vi "SCAN IM Stage Engine.vi"(0 "Notifier Name":string, 11 "COM Port":string[](array[string])) -> ()   [LabVIEW 2016]
uses:
  Stages Controls/Stage XY Control.ctl
  Stages Controls/Stage Status.ctl
  Stages Controls/Stage Notifier Element.ctl
  Stages Controls/Stage Actions.ctl
  <userlib>/Tango_DLL/Tango_DLL.lvlib
panel:
  out "Status":T1
  in  "Quit":bool
  in  "XY Control":T2
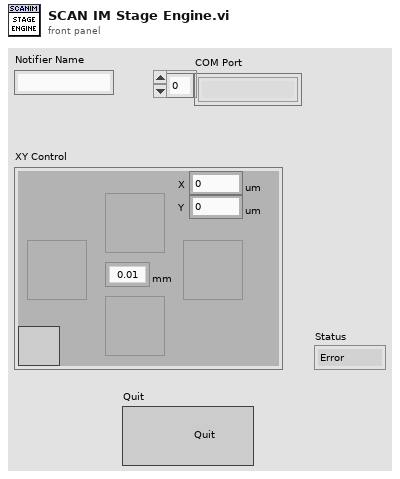
[diagram p1: front panel]
types:
  T1 = typedef "Stage Status.ctl" = enum16{"Error", "Abort", "Busy", "On Target"}
  T2 = typedef "Stage XY Control.ctl" = cluster{"Left":bool, "Right":bool, "Up":bool, "Down":bool, "Home":bool, "StageStep":enum16{"0.01", "0.02", "0.05", "0.1", "0.5", "1", "2", "5", "10", "20", "50", "100", "500", "1000", "2000", "5000"}, "Y":dbl, "X":dbl}
  T3 = typedef "Stage Notifier Element.ctl" = cluster{"Action":T4, "Axis":bool[], "Setpoint":dbl[], "Velocity":dbl, "Cmd Recvd?":bool, "Position":dbl[], "Status":T1, "Misc":variant}
  T4 = typedef "Stage Actions.ctl" = enum16{"Get Position", "MVR", "MOVE", "HALT", "ONTARGET", "ERROR", "REFERENCE", "INIT", "VELOCITY", "STATUS", "EXIT", "HOME", "ZEROPOS", "NANOPOS", "ANALOG", "QUIT"}
  T5 = cluster{"Left":bool, "Right":bool, "Up":bool, "Down":bool, "Home":bool, "StageStep":bool, "Y":bool, "X":bool}
  T6 = enum16{"0.01", "0.02", "0.05", "0.1", "0.5", "1", "2", "5", "10", "20", "50", "100", "500", "1000", "2000", "5000"}
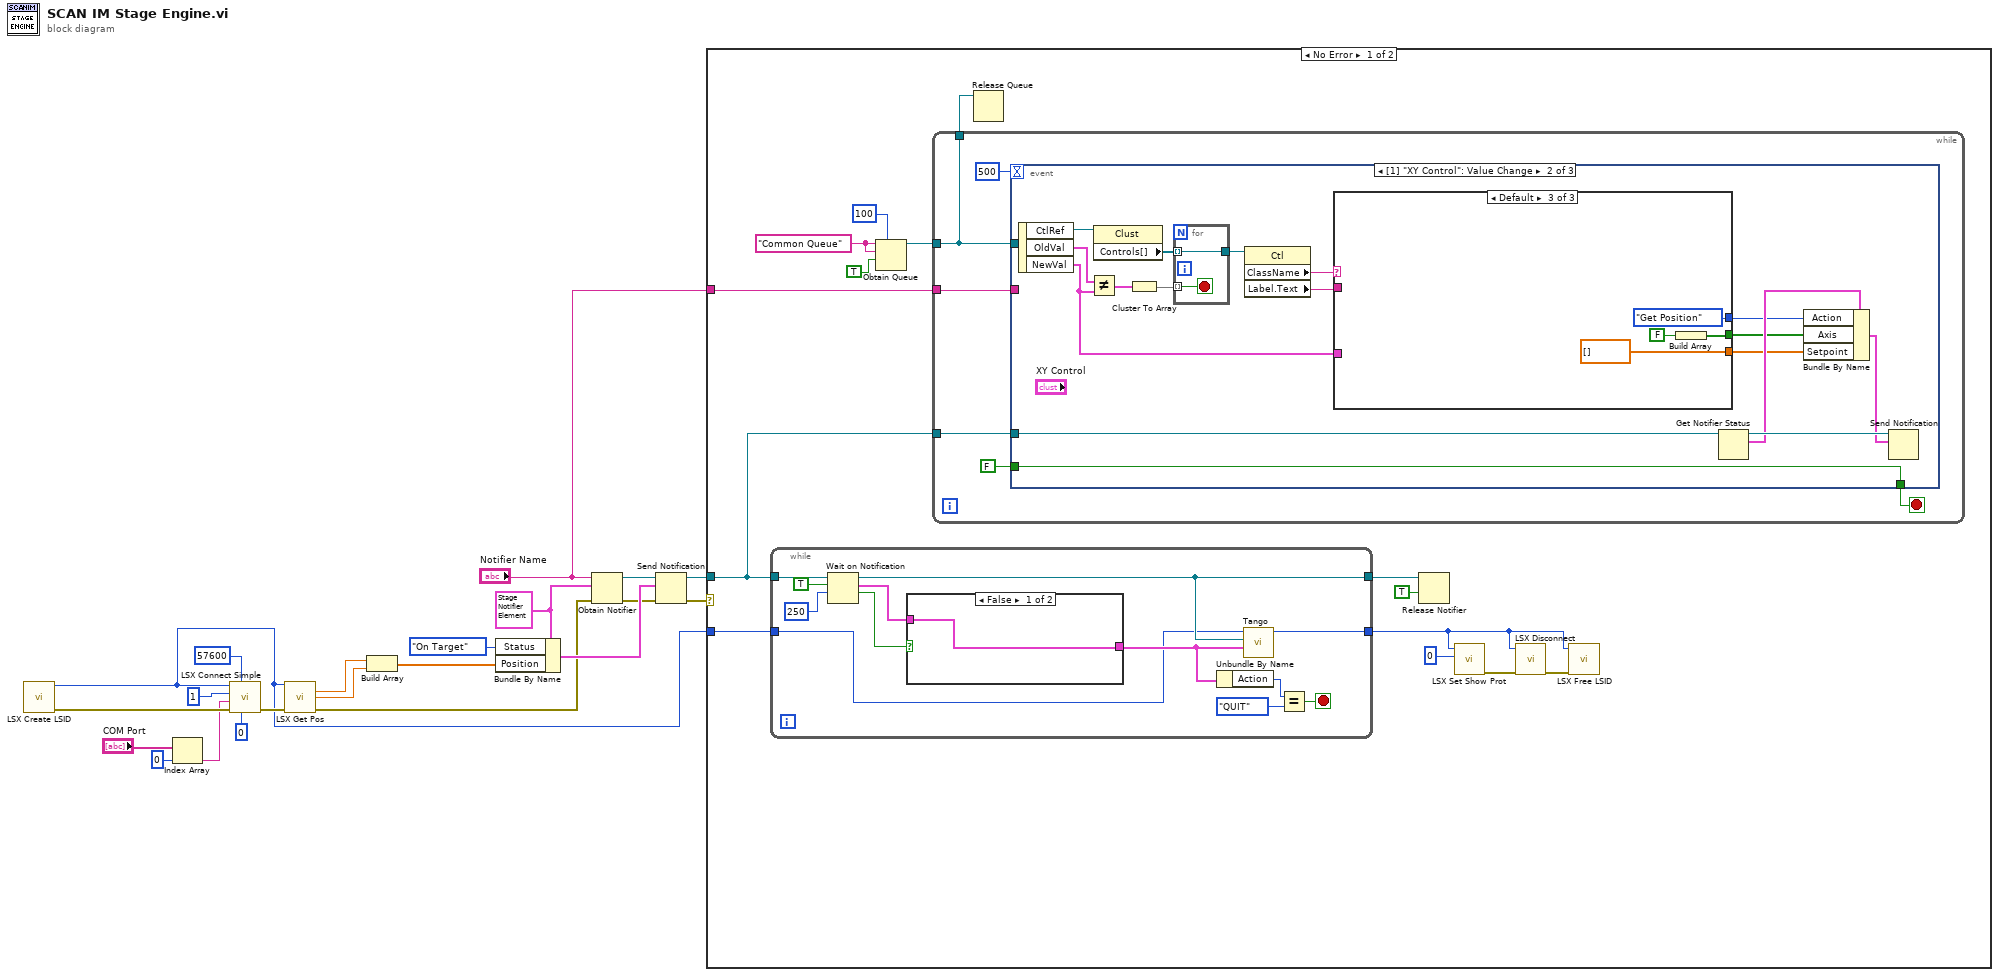
[diagram p0: block diagram]
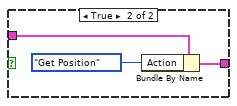
[diagram p2: hidden frame]
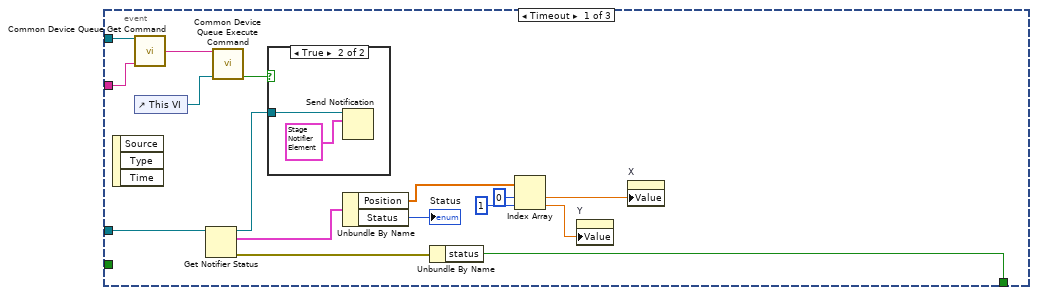
[diagram p3: hidden frame]
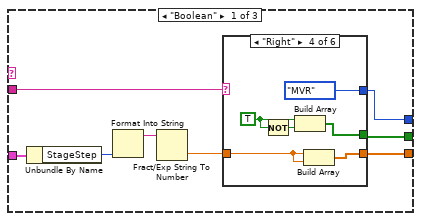
[diagram p5: hidden frame]
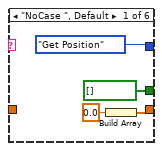
[diagram p6: hidden frame]
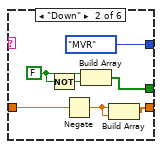
[diagram p7: hidden frame]
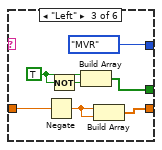
[diagram p8: hidden frame]
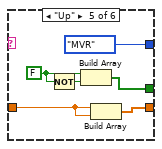
[diagram p9: hidden frame]
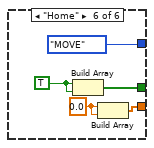
[diagram p10: hidden frame]
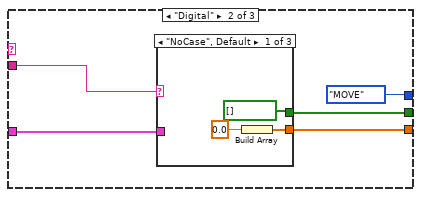
[diagram p11: hidden frame]
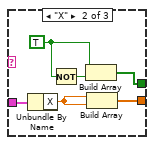
[diagram p12: hidden frame]
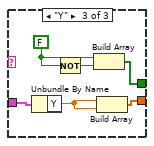
[diagram p13: hidden frame]
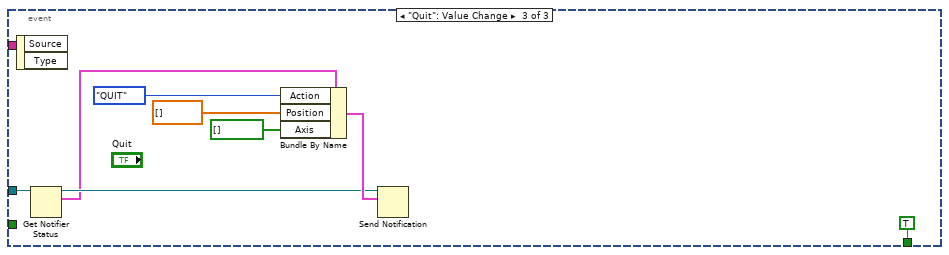
[diagram p14: hidden frame]
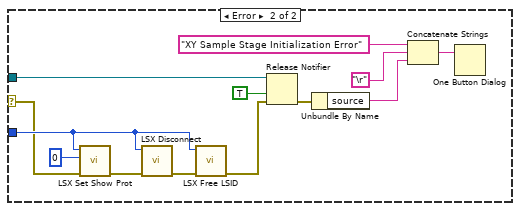
[diagram p15: hidden frame]
diagram:
  w20 = T3 {"Action"=enum."Get Position", "Axis"=[], "Setpoint"=[], "Velocity"=0.5, "Cmd Recvd?"=FALSE, "Position"=[], "Status"=enum."Abort", "Misc"=variant} ("Stage Status")
  n1 = call <userlib>:"LSX Create LSID.vi"() -> ("error out"=w15:errorcluster, "plLSID out"=w2:i32)  [unwired: 9 in, 1 out]
  n2 = Index Array(array="COM Port", index=0) -> (element=w5:string)
  n3 = call <userlib>:"LSX Connect Simple.vi"("bAShowProt"=0, "lABaudRate"=57600, "error in (no error)"=w15, "pcAComName"=w5, "lAnInterfaceType"=1, "lLSID"=w2) -> ("error out"=w9:errorcluster)  [unwired: 3 in, 2 out]
  n4 = call <userlib>:"LSX Get Pos.vi"("lLSID"=w2, "error in (no error)"=w9) -> ("pdX out"=w11:dbl, "pdY out"=w10:dbl, "error out"=w4:errorcluster)  [unwired: 8 in, 3 out]
  n5 = Build Array(w11, w10) -> (w17:dbl[])
  n6 = Bundle By Name(cluster=w20, "Status"=Stage_Status."On Target", "Position"=w17) -> (w19:T3)
  n7 = Obtain Notifier(name (unnamed)="Notifier Name", notification data type=w20, error in (no error)=w4) -> (notifier out=w21:refnum<notifier>, error out=w8:errorcluster)  [unwired: 1 in, 1 out]
  n8 = Send Notification(notification=w19, notifier=w21, error in (no error)=w8) -> (notifier out=w18:refnum<notifier>, error out=w3:errorcluster)
  n9 = case shown="No Error" w3 {
    selector: w3 -> [_ w171]
    tunnel: w18 -> [w34 w176]
    tunnel: w2 -> [w28 w172]
    tunnel: "Notifier Name" -> [w22 _]
    frame No Error {
      w25 = "Common Queue" ("Unique Notifier Name")
      n10 = while {
        tunnel: w28 -> [w36]
        tunnel: [w47] -> w29
        tunnel: w34 -> [w44]
        tunnel: [w37] -> w33
        stop <- w46 stop-if-true
        n11 = Wait on Notification(notifier=w44, ignore previous (F)=TRUE, timeout in ms (-1)=250) -> (notifier out=w37:refnum<notifier>, notification=w39:T3, timed out?=w40:bool)  [unwired: 1 in, 1 out]
        n12 = case shown="False" w40 {
          tunnel: w39 -> [w48 w51]
          tunnel: [w48 w49] -> w38
          frame False {
          }
          frame True {
            n13 = Bundle By Name(cluster=w51, "Action"=Stage_Actions."Get Position") -> (w49:T3)
          }
        }
        n14 = Unbundle By Name(w38) -> ("Action"=w42:T4)
        n15 = call "Tango.vi"("Stage Action"=w38, "Scan IM Notifier"=w37, "Tango Handle"=w36) -> ("Tango Handle"=w47:i32)  [unwired: 8 in]
        n16 = Equal?(x=w42, y=Stage_Actions."QUIT") -> (x = y?=w46:bool)
      }
      n17 = Obtain Queue(max queue size (-1, unlimited)=100, name (unnamed)=w25, element data type=w25, create if not found? (T)=TRUE) -> (queue out=w24:refnum<queue>)  [unwired: 1 in, 2 out]
      n18 = while {
        tunnel: w34 -> [w55]
        tunnel: w24 -> [w54]
        tunnel: [w54] -> w23
        tunnel: w22 -> [w53]
        stop <- w56 stop-if-true
        n19 = event shown="[1] \"XY Control\": Value Change" {
          selector: _ -> [_ _ _]
          dyn-events: _ -> [_ _ _]
          timeout: 500 -> [_ _ _]
          tunnel: [w73 w76 TRUE ("status")] -> w56
          tunnel: w55 -> [w72 w86 w166]
          tunnel: w54 -> [w62 _ _]
          tunnel: w53 -> [w61 _ _]
          tunnel: FALSE ("status") -> [_ w76 _]
          event Timeout {
            n20 = event-data() -> ()  [unwired: 1 in, 3 out]
            n21 = call "Common Device Queue Get Command.vi"("Common Queue"=w62, "Notifier Name"=w61) -> ("Command"=w60:string)  [unwired: 12 in, 1 out]
            n22 = control-ref of="This VI"() -> (w59:refnum<vi>)
            n23 = Get Notifier Status(notifier=w72) -> (notifier out=w58:refnum<notifier>, current notification=w71:T3, error out=w69:errorcluster)  [unwired: 1 in, 2 out]
            n24 = call "Common Device Queue Execute Command.vi"("Common Command"=w60, "VI Refnum"=w59) -> ("Quit?"=w63:bool)  [unwired: 12 in, 1 out]
            n25 = case shown="True" w63 {
              tunnel: w58 -> [_ w75]
              frame False {
              }
              frame True {
                n26 = Send Notification(notification=T3 {"Action"=enum."QUIT", "Axis"=[], "Setpoint"=[], "Velocity"=0.5, "Cmd Recvd?"=FALSE, "Position"=[], "Status"=enum."Error", "Misc"=variant} ("Stage Status"), notifier=w75) -> ()  [unwired: 1 in, 2 out]
              }
            }
            n27 = Unbundle By Name(w71) -> ("Position"=w70:dbl[], "Status"=→"Status":T1)
            n28 = Unbundle By Name(w69) -> ("status"=w73:bool)
            n29 = Index Array(array=w70, index #1=0 ("index"), index #2=1 ("index")) -> (element #1=w67:dbl, element #2=w66:dbl)
            n30 = property on="Y" class="DigNum (strict)"("Value"=w66) -> ()  [unwired: 2 in, 2 out]
            n31 = property on="X" class="DigNum (strict)"("Value"=w67) -> ()  [unwired: 2 in, 2 out]
          }
          event Value Change {
            n32 = event-data() -> ("CtlRef"=w91:refnum<vi>, "OldVal"=w92:T2, "NewVal"=w80:T2)  [unwired: 1 in]
            n33 = Not Equal?(x=w92, y=w80) -> (x != y?=w90:T5)
            n34 = property class="Clust"(reference=w91) -> ("Controls[]"=w88:refnum<vi>[])  [unwired: 1 in, 2 out]
            n35 = Cluster To Array(cluster=w90) -> (array=w89:bool[])
            n36 = for {
              tunnel: w89 -> [w161] mode=indexing
              tunnel: [w160] -> w87
              tunnel: w88 -> [w160] mode=indexing
              stop <- w161 stop-if-true
            }
            n37 = property class="Ctl"(reference=w87) -> ("ClassName"=w82:string, "Label.Text"=w81:string)  [unwired: 1 in, 2 out]
            n38 = case shown="Default" w82 {
              tunnel: w80 -> [w100 w139 _]
              tunnel: w81 -> [w95 w140 _]
              tunnel: [w96 w138 dbl[] []] -> w78
              tunnel: [w97 w137 w158] -> w79
              tunnel: [w93 Stage_Actions."MOVE" ("Action") Stage_Actions."Get Position" ("Action")] -> w77
              frame "Boolean" {
                n39 = Unbundle By Name(w100) -> ("StageStep"=w98:T6)
                n40 = Format Into String(w98) -> (resulting string=w99:string)  [unwired: 3 in, 1 out]
                n41 = Fract/Exp String To Number(string=w99) -> (number=w94:dbl)  [unwired: 3 in, 1 out]
                n42 = case shown="\"Right\"" w95 {
                  tunnel: [w102 w107 w114 w121 w127 w133] -> w96
                  tunnel: [bool[] [] w108 w115 w122 w128 w135] -> w97
                  tunnel: w94 -> [_ w111 w118 w120 w126 _]
                  tunnel: [Stage_Actions."Get Position" ("Action") Stage_Actions."MVR" ("Action") Stage_Actions."MVR" ("Action") Stage_Actions."MVR" ("Action") Stage_Actions."MVR" ("Action") Stage_Actions."MOVE" ("Action")] -> w93
                  frame "NoCase ", Default {
                    n43 = Build Array(0.0) -> (w102:dbl[])
                  }
                  frame "Down" {
                    w109 = FALSE
                    n44 = Not(x=w109) -> (.not. x?=w110:bool)
                    n45 = Negate(x=w111) -> (-x=w106:dbl)
                    n46 = Build Array(w109, w110) -> (w108:bool[])
                    n47 = Build Array(w106, w106) -> (w107:dbl[])
                  }
                  frame "Left" {
                    w116 = TRUE
                    n48 = Negate(x=w118) -> (-x=w113:dbl)
                    n49 = Not(x=w116) -> (.not. x?=w117:bool)
                    n50 = Build Array(w116, w117) -> (w115:bool[])
                    n51 = Build Array(w113, w113) -> (w114:dbl[])
                  }
                  frame "Right" {
                    w123 = TRUE
                    n52 = Not(x=w123) -> (.not. x?=w124:bool)
                    n53 = Build Array(w123, w124) -> (w122:bool[])
                    n54 = Build Array(w120, w120) -> (w121:dbl[])
                  }
                  frame "Up" {
                    w129 = FALSE
                    n55 = Not(x=w129) -> (.not. x?=w130:bool)
                    n56 = Build Array(w129, w130) -> (w128:bool[])
                    n57 = Build Array(w126, w126) -> (w127:dbl[])
                  }
                  frame "Home" {
                    w132 = 0.0
                    w134 = TRUE
                    n58 = Build Array(w134, w134) -> (w135:bool[])
                    n59 = Build Array(w132, w132) -> (w133:dbl[])
                  }
                }
              }
              frame "Digital" {
                n60 = case shown="\"NoCase\", Default" w140 {
                  tunnel: [bool[] [] w148 w153] -> w137
                  tunnel: w139 -> [_ w147 w152]
                  tunnel: [w141 w146 w151] -> w138
                  frame "NoCase", Default {
                    n61 = Build Array(0.0 ("Y axis (mm)")) -> (w141:dbl[])
                  }
                  frame "X" {
                    w149 = TRUE
                    n62 = Unbundle By Name(w147) -> ("X"=w145:dbl)
                    n63 = Not(x=w149) -> (.not. x?=w144:bool)
                    n64 = Build Array(w149, w144) -> (w148:bool[])
                    n65 = Build Array(w145, w145) -> (w146:dbl[])
                  }
                  frame "Y" {
                    w155 = FALSE
                    n66 = Unbundle By Name(w152) -> ("Y"=w150:dbl)
                    n67 = Not(x=w155) -> (.not. x?=w154:bool)
                    n68 = Build Array(w155, w154) -> (w153:bool[])
                    n69 = Build Array(w150, w150) -> (w151:dbl[])
                  }
                }
              }
              frame Default {
                n70 = Build Array(FALSE) -> (w158:bool[])
              }
            }
            n71 = Get Notifier Status(notifier=w86) -> (notifier out=w85:refnum<notifier>, current notification=w84:T3)  [unwired: 1 in, 3 out]
            n72 = Bundle By Name(cluster=w84, "Action"=w77, "Axis"=w79, "Setpoint"=w78) -> (w83:T3)
            n73 = Send Notification(notification=w83, notifier=w85) -> ()  [unwired: 1 in, 2 out]
          }
          event "Quit": Value Change {
            n74 = event-data() -> ()  [unwired: 1 in, 2 out]
            n75 = Get Notifier Status(notifier=w166) -> (notifier out=w164:refnum<notifier>, current notification=w163:T3)  [unwired: 1 in, 3 out]
            n76 = Bundle By Name(cluster=w163, "Action"=Stage_Actions."QUIT", "Position"=dbl[] [], "Axis"=bool[] []) -> (w167:T3)
            n77 = Send Notification(notification=w167, notifier=w164) -> ()  [unwired: 1 in, 2 out]
          }
        }
      }
      n78 = Release Queue(queue=w23) -> ()  [unwired: 2 in, 3 out]
      n79 = Release Notifier(notifier=w33, force destroy? (F)=TRUE) -> ()  [unwired: 1 in, 3 out]
      n80 = call <userlib>:"LSX Set Show Prot.vi"("bShowProt"=0, "lLSID"=w29) -> ("error out"=w31:errorcluster)  [unwired: 8 in, 1 out]
      n81 = call <userlib>:"LSX Disconnect.vi"("error in (no error)"=w31, "lLSID"=w29) -> ("error out"=w32:errorcluster)  [unwired: 8 in, 1 out]
      n82 = call <userlib>:"LSX Free LSID.vi"("error in (no error)"=w32, "lLSID"=w29) -> ()  [unwired: 8 in, 2 out]
    }
    frame Error {
      n83 = call <userlib>:"LSX Set Show Prot.vi"("error in (no error)"=w171, "bShowProt"=0, "lLSID"=w172) -> ("error out"=w174:errorcluster)  [unwired: 7 in, 1 out]
      n84 = call <userlib>:"LSX Disconnect.vi"("error in (no error)"=w174, "lLSID"=w172) -> ("error out"=w175:errorcluster)  [unwired: 8 in, 1 out]
      n85 = call <userlib>:"LSX Free LSID.vi"("error in (no error)"=w175, "lLSID"=w172) -> ("error out"=w170:errorcluster)  [unwired: 8 in, 1 out]
      n86 = Release Notifier(notifier=w176, force destroy? (F)=TRUE, error in (no error)=w170) -> (error out=w181:errorcluster)  [unwired: 2 out]
      n87 = Unbundle By Name(w181) -> ("source"=w178:string)
      n88 = Concatenate Strings("XY Sample Stage Initialization Error", "\r", w178) -> (w177:string)
      n89 = One Button Dialog(message=w177) -> ()  [unwired: 1 in, 1 out]
    }
  }
